vi "CANsub_Check_Stopped.vi"(8 "error in (no error)":errorcluster, 11 "response":string) -> (0 "error out":errorcluster, 2 "ok":bool, 3 "state":string)   [LabVIEW 2021, in "CANsub_Common.lvlib"]
doc: "Checks from the GET channel response that the CAN channel is stopped, so no other client owns it. Error 5002: channel busy (close webCAN or the other client; a client that did not close: curl -sk -X DELETE https://<host>/api/can/<ch>/ws)."
uses:
  CANsub_Common.lvlib
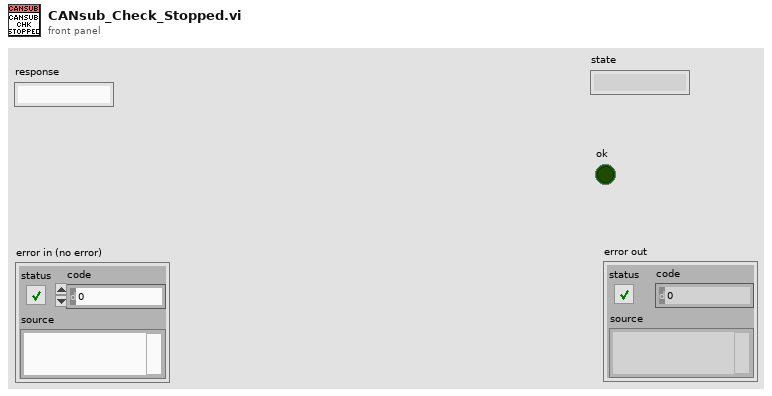
[diagram p1: front panel]
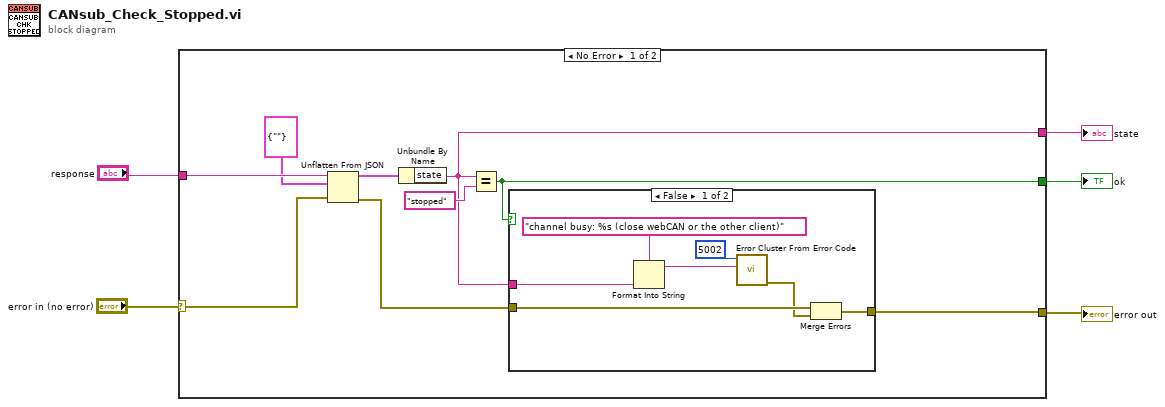
[diagram p0: block diagram]
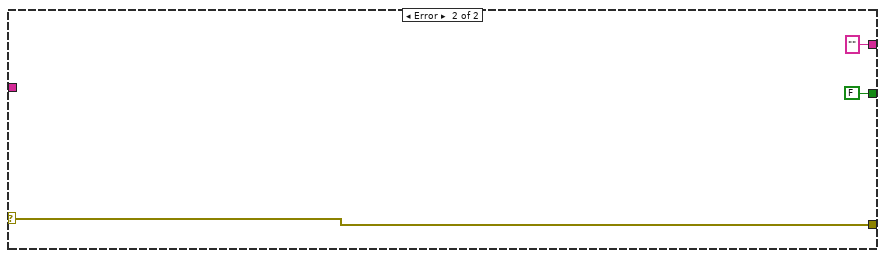
[diagram p3: hidden frame]
diagram:
  n1 = case shown="No Error" "error in (no error)" {
    selector: "error in (no error)" -> [w12 w25]
    tunnel: [w7 w25] -> w5
    tunnel: "response" -> [w14 _]
    tunnel: [w9 FALSE] -> w2
    tunnel: [w6 "" ("state")] -> w1
    frame No Error {
      n2 = Unflatten From JSON(JSON string=w14, type and defaults=cluster{"state":string} {"state"=""}, error in (no error)=w12) -> (value=w11:cluster{"state":string}, error out=w8:errorcluster)  [unwired: 4 in]
      n3 = Unbundle By Name(w11) -> ("state"=w6:string)
      n4 = Equal?(x=w6, y="stopped") -> (x = y?=w9:bool)
      n5 = case shown="False" w9 {
        tunnel: [w15 w22] -> w7
        tunnel: w8 -> [w17 w22]
        tunnel: w6 -> [w20 _]
        frame False {
          n6 = Format Into String(format string="channel busy: %s (close webCAN or the other client)", w20) -> (resulting string=w18:string)  [unwired: 2 in, 1 out]
          n7 = call <vilib>:"Error Cluster From Error Code.vi"("error message (\"\")"=w18, "error code (0)"=5002) -> ("error out"=w16:errorcluster)  [unwired: 7 in]
          n8 = Merge Errors(w17, w16) -> (w15:errorcluster)
        }
        frame True {
        }
      }
    }
    frame Error {
    }
  }
  "error out" <- w5
  "state" <- w1
  "ok" <- w2
